vi "Compute Possible Connections.vi"(8 "error in":errorcluster, 11 "ni-switch custom device in":T3 format="%.0x") -> (0 "error out":errorcluster, 1 "existing connections":T1[](array[typedef]), 2 "possible connections":T2[](array[typedef]), 3 "ni-switch custom device out":T3 format="%.0x")   [LabVIEW 2020, in "NI-SWITCH Scripting.lvlib"]
uses:
  NI-SWITCH Scripting.lvlib
  <vilib>/NI VeriStand/Custom Device API/Custom Device Item Ref.ctl
  Shared/Routing and Faulting Hardware API/Types/Possible Connections for Endpoint.ctl
  Shared/Routing and Faulting Hardware API/Types/Connection.ctl
  Shared/Routing and Faulting Hardware API/Routing and Faulting Hardware API.lvlib
  <vilib>/NI VeriStand/Custom Device API/Custom Device API.lvlib
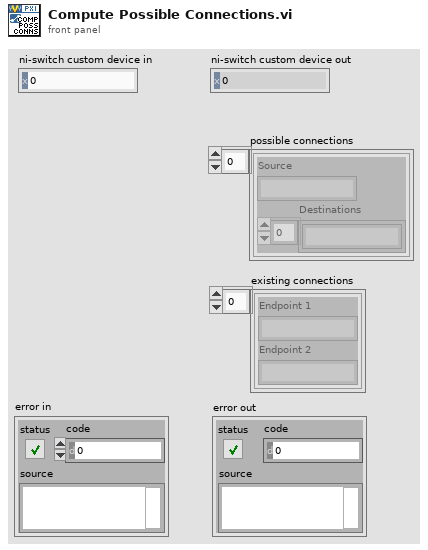
[diagram p1: front panel]
types:
  T1 = typedef "Routing and Faulting Hardware API.lvlib/Connection.ctl" = cluster{"Endpoint 1":string, "Endpoint 2":string}
  T2 = typedef "Routing and Faulting Hardware API.lvlib/Possible Connections for Endpoint.ctl" = cluster{"Source":string, "Destinations":string[]}
  T3 = typedef "Custom Device API.lvlib/Custom Device Item Ref.ctl" = u64
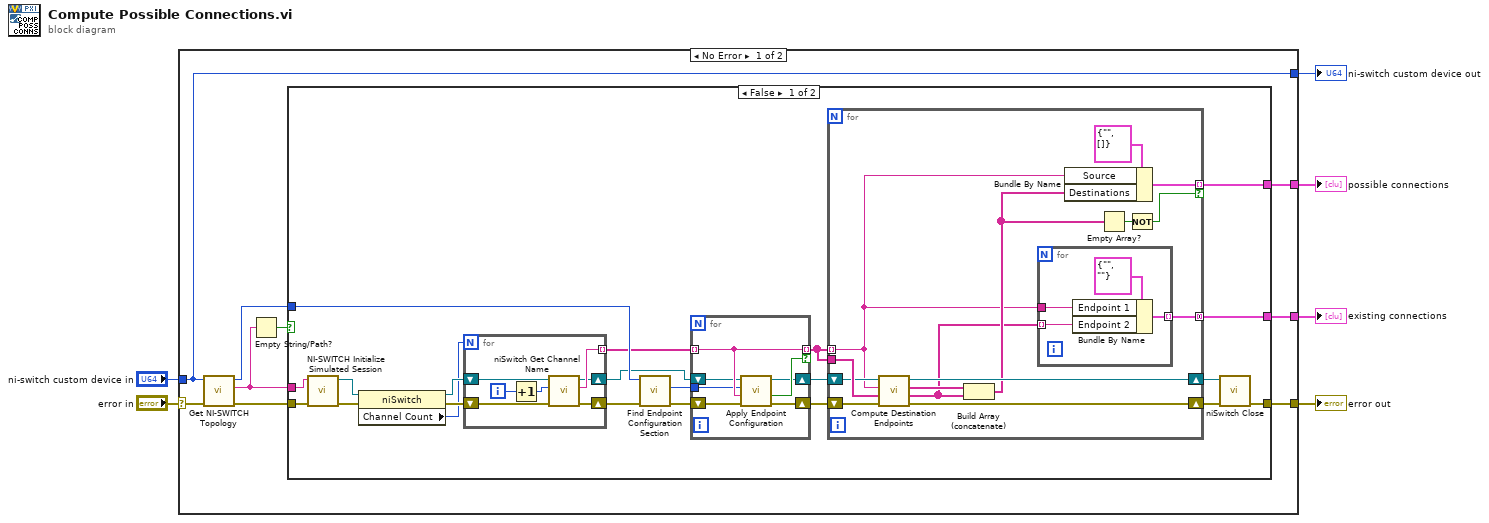
[diagram p0: block diagram]
diagram:
  n1 = case shown="No Error" "error in" {
    selector: "error in" -> [w9 w71]
    tunnel: [w15 w71] -> w6
    tunnel: "ni-switch custom device in" -> [w10 w70]
    tunnel: [w10 w70] -> w4
    tunnel: [w12 _] -> w2
    tunnel: [w7 _] -> w1
    frame No Error {
      n2 = call "Get NI-SWITCH Topology.vi"("error in"=w9, "ni-switch custom device in"=w10) -> ("error out"=w13:errorcluster, "topology"=w11:string, "ni-switch custom device out"=w14:T3)  [unwired: 7 in]
      n3 = Empty String/Path?(string/path=w11) -> (empty?=w8:bool)
      n4 = case shown="False" w8 {
        tunnel: [w18 w69] -> w15
        tunnel: w11 -> [w28 _]
        tunnel: w14 -> [w31 _]
        tunnel: w13 -> [w29 w69]
        tunnel: [w33 _] -> w12
        tunnel: [w16 _] -> w7
        frame False {
          n5 = call "NI-SWITCH Initialize Simulated Session.vi"("error in (no error)"=w29, "topology"=w28) -> ("error out"=w24:errorcluster, "NI-SWITCH session"=w23:refnum<k15>)  [unwired: 8 in]
          n6 = property class="niSwitch"(reference=w23, error in=w24) -> (reference out=w27:refnum<k15>, error out=w26:errorcluster, "Channel Count"=w25:i32)
          n7 = for {
            N: w25 -> [_]
            tunnel: [w41] -> w20 mode=indexing
            shift-right: [w40] -> w21
            shift-left: w26 -> [w42]
            shift-right: [w37] -> w22
            shift-left: w27 -> [w43]
            i -> [w39]
            n8 = Increment(x=w39) -> (x+1=w38:i32)
            n9 = call <instrlib>:"niSwitch Get Channel Name.vi"("error in (no error)"=w42, "index (1)"=w38, "instrument handle"=w43) -> ("error out"=w40:errorcluster, "channel string"=w41:string, "instrument handle out"=w37:refnum<k15>)  [unwired: 6 in]
          }
          n10 = call "Find Endpoint Configuration Section.vi"("error in"=w21, "ni-switch custom device in"=w31) -> ("error out"=w32:errorcluster, "endpoint configuration"=w30:T3)  [unwired: 7 in, 1 out]
          n11 = for {
            tunnel: [w47] -> w36 mode=indexing if=w50
            tunnel: w20 -> [w47] mode=indexing
            tunnel: w30 -> [w45]
            shift-right: [w48] -> w35
            shift-left: w32 -> [w49]
            shift-right: [w44] -> w34
            shift-left: w22 -> [w46]
            n12 = call "Apply Endpoint Configuration.vi"("error in"=w49, "endpoint"=w47, "endpoint configuration in"=w45, "instrument handle in"=w46) -> ("error out"=w48:errorcluster, "endpoint addressable?"=w50:bool, "instrument handle out"=w44:refnum<k15>)  [unwired: 4 in, 1 out]
          }
          n13 = for {
            tunnel: w36 -> [w53] mode=indexing
            tunnel: w36 -> [w64]
            shift-right: [w62] -> w19
            shift-left: w35 -> [w63]
            shift-right: [w61] -> w17
            shift-left: w34 -> [w55]
            tunnel: [w57] -> w33 mode=indexing if=w56
            tunnel: [w51] -> w16 mode=concatenating
            n14 = call "Compute Destination Endpoints.vi"("error in"=w63, "endpoints"=w64, "source endpoint"=w53, "instrument handle in"=w55) -> ("error out"=w62:errorcluster, "existing destinations"=w52:string[], "available destinations"=w58:string[], "instrument handle out"=w61:refnum<k15>)  [unwired: 4 in]
            n15 = Build Array (concatenate)(w58, w52) -> (w54:string[])
            n16 = for {
              tunnel: w53 -> [w67]
              tunnel: w52 -> [w66] mode=indexing
              tunnel: [w65] -> w51 mode=indexing
              n17 = Bundle By Name(cluster=T1 {"Endpoint 1"="", "Endpoint 2"=""} ("Connection"), "Endpoint 1"=w67, "Endpoint 2"=w66) -> (w65:T1)
            }
            n18 = Bundle By Name(cluster=T2 {"Source"="", "Destinations"=[]} ("Possible Connections for Endpoint"), "Source"=w53, "Destinations"=w54) -> (w57:T2)
            n19 = Empty Array?(array=w54) -> (empty?=w59:bool)
            n20 = Not(x=w59) -> (.not. x?=w56:bool)
          }
          n21 = call <instrlib>:"niSwitch Close.vi"("error in (no error)"=w19, "instrument handle"=w17) -> ("error out"=w18:errorcluster)  [unwired: 9 in]
        }
        frame True {
        }
      }
    }
    frame Error {
    }
  }
  "error out" <- w6
  "ni-switch custom device out" <- w4
  "possible connections" <- w2
  "existing connections" <- w1
